vi "SelectObject Wrapper Template.vi"(0 "hdc":u64, 5 "h":u64, 11 "error in":errorcluster) -> (4 "previous object":u64, 15 "error out":errorcluster)   [LabVIEW 2020]
doc: "Selects the GDI object h (a bitmap, pen, brush ...) into the device context hdc through gdi32.dll SelectObject (stdcall, called in any thread) and returns the object it replaced - select that one back before deleting h. When error in carries an error the DLL is not called. Generated by scripts\\Build Win32 Wrappers.vi - do not edit by hand, rebuild it."
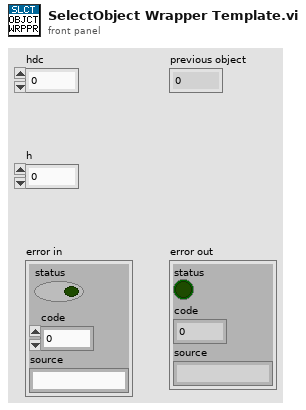
[diagram p1: front panel]
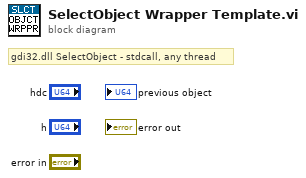
[diagram p0: block diagram]
diagram:
  # "gdi32.dll SelectObject - stdcall, any thread"
